vi "Handle Last Ack Core.vi"(4 "error in (no error)":errorcluster, 6 "Last Ack":refnum<class "Last Ack.lvclass">, 7 "DAQ Timed SPIM in":refnum<class "DAQ Timed SPIM.lvclass">) -> (0 "error out":errorcluster, 3 "DAQ Timed SPIM out":refnum<class "DAQ Timed SPIM.lvclass">)   [LabVIEW 2020, in "DAQ Timed SPIM.lvlib" / "DAQ Timed SPIM.lvclass"]
doc: "(<B>Filename</B>: Actor Framework.lvlib:Actor.lvclass:Handle Last Ack Core.vi)\n\nDefines how the caller actor responds to the Last Ack message from a nested actor. The Last Ack message is the final message a nested actor sends to its caller before it shuts down. The message contains information about the final state of the nested actor.\n\nBy default, this method does nothing except return any error the nested actor sent. A descendant class may override this method to define behavior."
uses:
  DAQ Timed SPIM.lvclass
  <vilib>/ActorFramework/LastAck/Last Ack.lvclass
  DAQ Timed SPIM.lvclass/DAQ Timed SPIM.ctl
  <vilib>/ActorFramework/Actor/Actor.lvclass
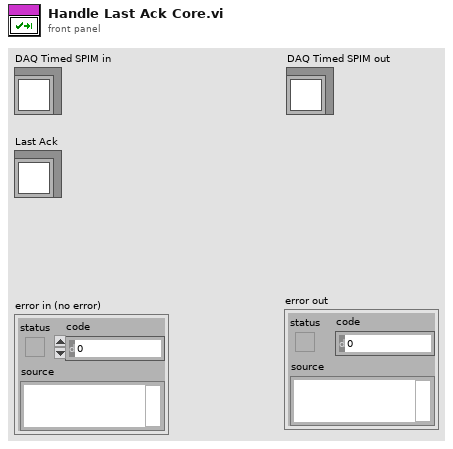
[diagram p1: front panel]
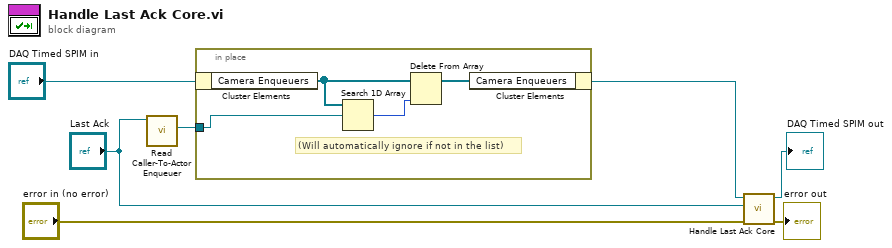
[diagram p0: block diagram]
diagram:
  n1 = call <vilib>:"Read Caller-To-Actor Enqueuer.vi"("Last Ack"="Last Ack") -> ("Caller-to-Actor Enqueuer"=w3:refnum<class "Message Enqueuer.lvclass">)  [unwired: 10 in]
  n2 = in-place {
    in-place-border: w3 -> [w11]
    # "(Will automatically ignore if not in the list)"
    n3 = in-place-cluster #1("DAQ Timed SPIM in") -> ("Camera Enqueuers"=w10:refnum<class "Message Enqueuer.lvclass">[])
    n4 = Search 1D Array(1D array=w10, element=w11) -> (index of element=w8:i32)  [unwired: 1 in]
    n5 = Delete From Array(array=w10, index=w8) -> (array with subset deleted=w9:refnum<class "Message Enqueuer.lvclass">[])  [unwired: 1 in, 1 out]
    n6 = in-place-cluster #1("Camera Enqueuers"=w9) -> (w4:refnum<class "DAQ Timed SPIM.lvclass">)
  }
  n7 = call-parent "Handle Last Ack Core.vi"("error in (no error)"="error in (no error)", "Last Ack"="Last Ack", "Actor in"=w4) -> ("error out"=→"error out":errorcluster, "Actor out"=→"DAQ Timed SPIM out":refnum<class "DAQ Timed SPIM.lvclass">)  [unwired: 3 in]
